vi "Sleep Test.vi"() -> ()   [LabVIEW 2013]
uses:
  Source/VIs/Public/Time/Get Clock Time (timespec).vi
  Source/VIs/Public/Time/Nanosleep Absolute (timespec).vi
  Source/Linux RT Utilities.lvlib
panel:
  out "Loop 1":i32
  out "Loop 2":i32
  in  "stop":bool
  in  "Period (ns)":i64=1000000 format="%#.3p"
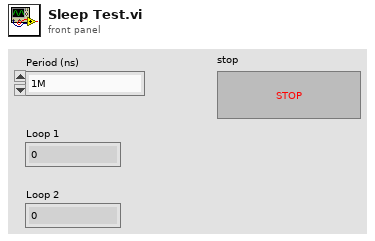
[diagram p1: front panel]
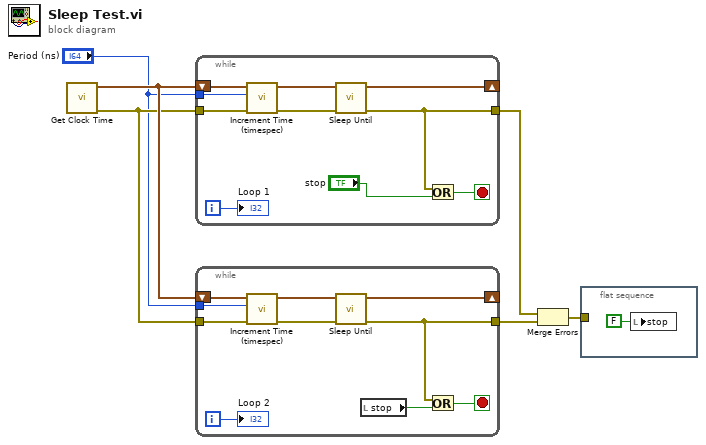
[diagram p0: block diagram]
diagram:
  n1 = call-poly "Get Clock Time.vi"() -> ("error out"=w3:errorcluster, "timespec"=w4:cluster{"sec":u64, "nsec":u64})  [unwired: 10 in]
  n2 = while {
    tunnel: w3 -> [w15]
    shift-right: [w8] -> _
    shift-left: w4 -> [w16]
    tunnel: "Period (ns)" -> [w14]
    tunnel: [w10] -> w1
    i -> [w11]
    stop <- w12 stop-if-true
    n3 = call "Increment Time (timespec).vi"("error in (no error)"=w15, "nanos offset"=w14, "timespec in"=w16) -> ("error out"=w13:errorcluster, "timespec out"=w9:cluster{"sec":u64, "nsec":u64})  [unwired: 7 in]
    n4 = call-poly "Sleep Until.vi"("error in (no error)"=w13, "sleep until (timespec)"=w9) -> ("error out"=w10:errorcluster, "current time (timspec)"=w8:cluster{"sec":u64, "nsec":u64})  [unwired: 8 in]
    n5 = Or(x=w10, y="stop") -> (x .or. y?=w12:bool)
    "Loop 1" <- w11
  }
  n6 = while {
    tunnel: w3 -> [w25]
    shift-right: [w17] -> _
    shift-left: w4 -> [w26]
    tunnel: "Period (ns)" -> [w24]
    tunnel: [w19] -> w6
    i -> [w21]
    stop <- w22 stop-if-true
    n7 = call "Increment Time (timespec).vi"("error in (no error)"=w25, "nanos offset"=w24, "timespec in"=w26) -> ("error out"=w23:errorcluster, "timespec out"=w18:cluster{"sec":u64, "nsec":u64})  [unwired: 7 in]
    n8 = call-poly "Sleep Until.vi"("error in (no error)"=w23, "sleep until (timespec)"=w18) -> ("error out"=w19:errorcluster, "current time (timspec)"=w17:cluster{"sec":u64, "nsec":u64})  [unwired: 8 in]
    n9 = local read "stop"() -> (w20:bool)
    n10 = Or(x=w19, y=w20) -> (x .or. y?=w22:bool)
    "Loop 2" <- w21
  }
  n11 = Merge Errors(w1, w6) -> (w5:errorcluster)
  n12 = flat-sequence {
    tunnel: w5 -> [_]
    frame #0 {
      n13 = local write "stop"(FALSE ("stop")) -> ()
    }
  }
